vi "BSD PNG Burst.vi"(6 "Color":u32[](array[numeric]), 7 "R Level":dbl[](array[numeric]), 8 "error in":errorcluster, 9 "BC1":cluster{"B region#":i32, "Date":string}, 10 "BSE path":string, 11 "Time Graph":cluster{"time":dbl[], "current":dbl[]}[](graph)) -> (0 "error out":errorcluster)   [LabVIEW 2018]
panel:
  out "Path":path
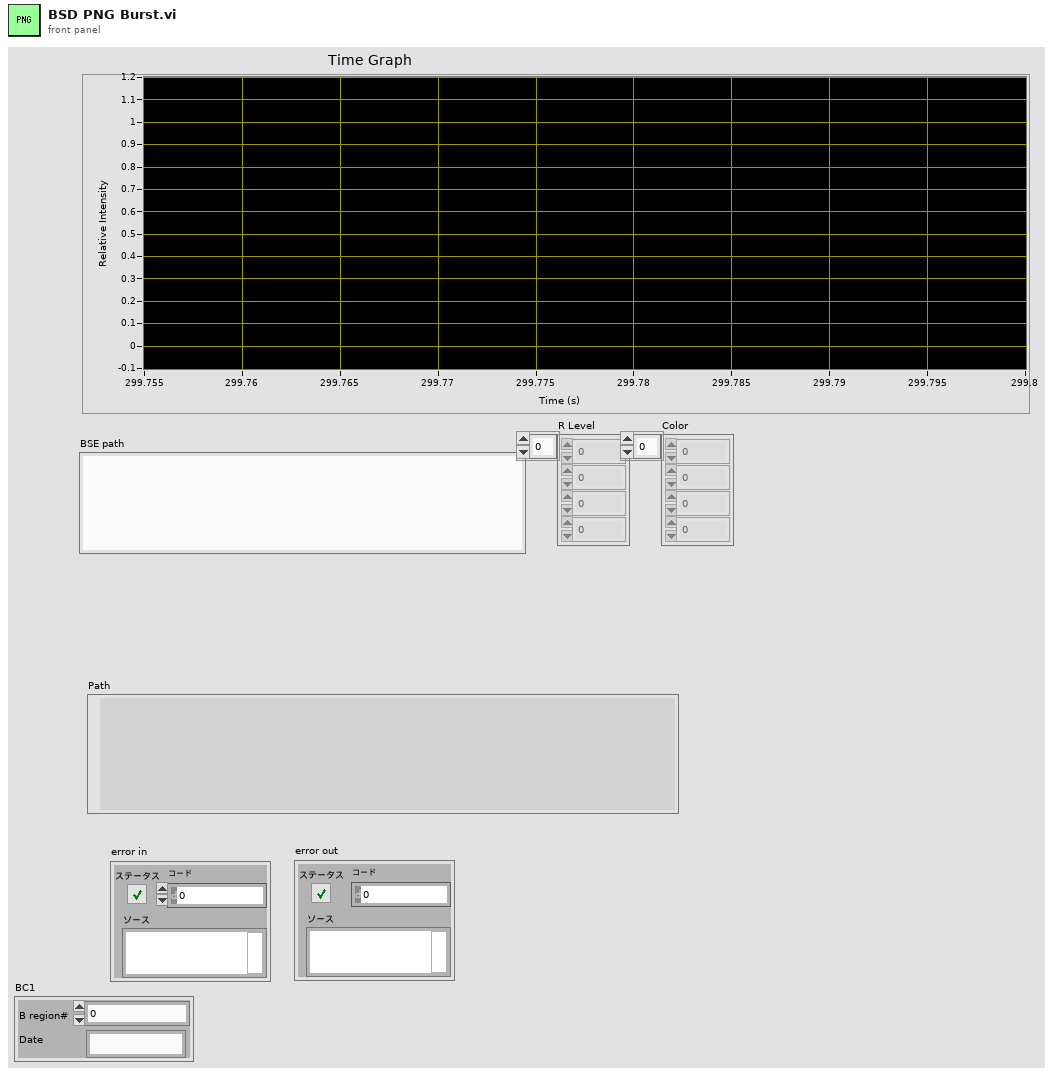
[diagram p1: front panel]
types:
  T1 = typedef "imagedata.ctl" = cluster{"image type":i32, "image depth":i32, "image":u8[], "mask":u8[], "colors":u32[], "Rectangle":cluster{"left":i16, "top":i16, "right":i16, "bottom":i16}}
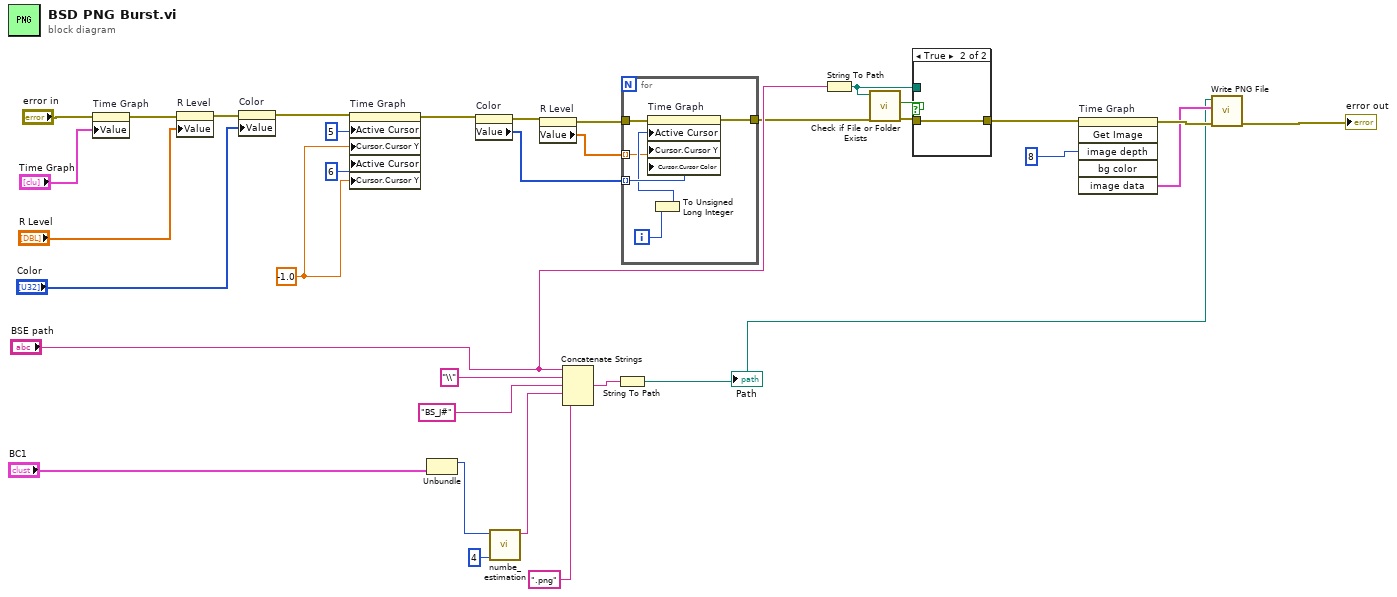
[diagram p0: block diagram]
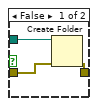
[diagram p2: hidden frame]
diagram:
  w8 = -1.0 ("画像深度")
  n1 = property on="Time Graph" class="XYGraph (strict)"(error in="error in", "Value"="Time Graph") -> (error out=w18:errorcluster)  [unwired: 1 in, 1 out]
  n2 = property on="R Level" class="Arr (strict)"(error in=w18, "Value"="R Level") -> (error out=w17:errorcluster)  [unwired: 1 in, 1 out]
  n3 = property on="Color" class="Arr (strict)"(error in=w17, "Value"="Color") -> (error out=w12:errorcluster)  [unwired: 1 in, 1 out]
  n4 = property on="Time Graph" class="XYGraph (strict)"(error in=w12, "Active Cursor"=u32 5 ("アクティブカーソル"), "Cursor.Cursor Y"=w8, "Active Cursor"=u32 6 ("アクティブカーソル"), "Cursor.Cursor Y"=w8) -> (error out=w11:errorcluster)  [unwired: 1 in, 1 out]
  n5 = Unbundle("BC1") -> ("B region#"=w25:i32)  [unwired: 1 out]
  n6 = property on="Color" class="Arr (strict)"(error in=w11) -> (error out=w7:errorcluster, "Value"=w13:u32[])  [unwired: 1 in, 1 out]
  n7 = call "numbe_estimation.vi"("桁数"=4, "数値"=w25) -> ("数値文字列"=w22:string)  [unwired: 9 in]
  n8 = property on="R Level" class="Arr (strict)"(error in=w7) -> (error out=w15:errorcluster, "Value"=w14:dbl[])  [unwired: 1 in, 1 out]
  n9 = Concatenate Strings("BSE path", "\\" ("文字列"), "BS_J#" ("文字列"), w22, ".png" ("文字列")) -> (w28:string)
  n10 = String To Path(string=w28) -> (path=w30:path)
  "Path" <- w30
  n11 = for {
    tunnel: w15 -> [w40]
    tunnel: [w39] -> w2
    tunnel: w13 -> [w38] mode=indexing
    tunnel: w14 -> [w35] mode=indexing
    i -> [w37]
    n12 = To Unsigned Long Integer(number=w37) -> (unsigned 32bit integer=w36:u32)
    n13 = property on="Time Graph" class="XYGraph (strict)"(error in=w40, "Active Cursor"=w36, "Cursor.Cursor Y"=w35, "Cursor.Cursor Color"=w38) -> (error out=w39:errorcluster)  [unwired: 1 in, 1 out]
  }
  n14 = String To Path(string="BSE path") -> (path=w6:path)
  n15 = call <vilib>:"Check if File or Folder Exists.vi"("error in (no error)"=w2, "path"=w6) -> ("error out"=w4:errorcluster, "file or folder exists?"=w5:bool)  [unwired: 7 in, 1 out]
  n16 = case shown="True" w5 {
    tunnel: w6 -> [w43 _]
    tunnel: w4 -> [w42 w44]
    tunnel: [w41 w44] -> w1
    frame False {
      n17 = Create Folder(path (use dialog)=w43, error in=w42) -> (error out=w41:errorcluster)  [unwired: 1 in, 2 out]
    }
    frame True {
    }
  }
  n18 = invoke on="Time Graph" class="XYGraph （指定）" method="Get Image"(error in=w1, "image depth"=8 ("画像深度")) -> (error out=w34:errorcluster, "image data"=w32:T1)  [unwired: 4 in, 4 out]
  n19 = call <vilib>:"Write PNG File.vi"("error in (no error)"=w34, "image data"=w32, "path to PNG file"=w30) -> ("error out"=→"error out":errorcluster)  [unwired: 7 in, 1 out]
